vi "UNITTEST-JSON-RPC-Parse-Error.vi"(8 "error in (no error)":errorcluster) -> (0 "error out":errorcluster)   [LabVIEW 2019]
uses:
  <vilib>/addons/_JKI Toolkits/Caraya/classes/Assert/Assert Not Error.vi
  <vilib>/addons/_JKI Toolkits/Caraya/classes/Assert/Assert False.vi
  JSON-RPC/JSON-RPC.lvlib
  <vilib>/addons/_JKI Toolkits/Caraya/classes/Assert/Assert.lvclass
  <vilib>/addons/_JKI Toolkits/Caraya/classes/Test/Test.lvclass
  <vilib>/JDP Science/JSONtext/JSONtext.lvlib
panel:
  out "Array":string[](array[string])
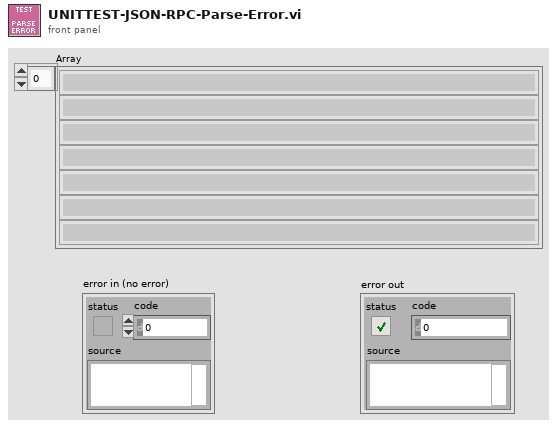
[diagram p1: front panel]
types:
  T1 = cluster{"error in (no error)":errorcluster, "id":string, "<JSON>":string, "response":string}[]
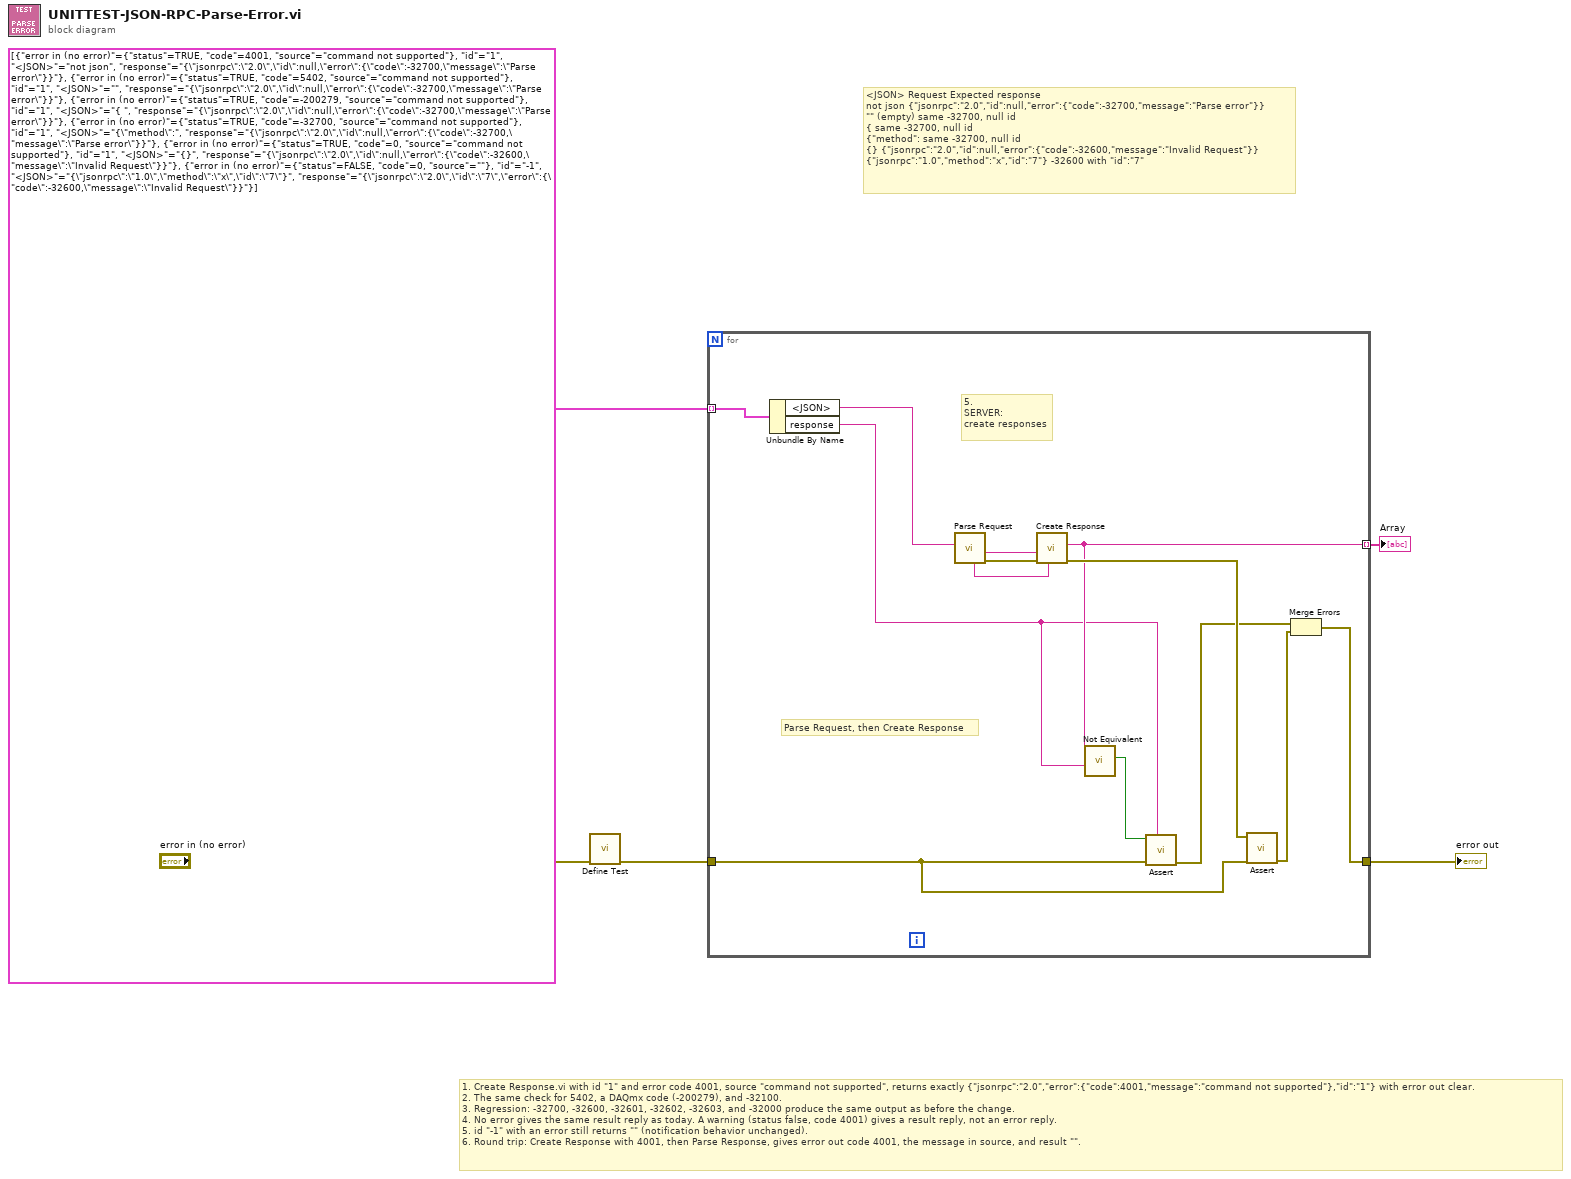
[diagram p0: block diagram]
diagram:
  # "<JSON> Request\tExpected response\nnot json\t{\"jsonrpc\":\"2.0\",\"id\":null,\"error\":{\"code\":-32700,\"message\":\"Parse error\"}}\n\"\" (empty)\tsame -32700, null id\n{\tsame -32700, null id\n{\"method\":\tsame -32700, null id\n{}\t{\"jsonrpc\":\"2.0\",\"id\":null,\"error\":{\"code\":-32600,\"message\":\"Invalid Request\"}}\n{\"jsonrpc\":\"1.0\",\"method\":\"x\",\"id\":\"7\"}\t-32600 with \"id\":\"7\""
  # "1. Create Response.vi with id \"1\" and error code 4001, source \"command not supported\", returns exactly {\"jsonrpc\":\"2.0\",\"error\":{\"code\":4001,\"message\":\"command not supported\"},\"id\":\"1\"} with error out clear.\n2. The same check for 5402, a DAQmx code (-200279), and -32100.\n3. Regression: -32700, -32600, -32601, -32602, -32603, and -32000 produce the same output as before the change.\n4. No error gives the same result reply as today. A warning (status false, code 4001) gives a result reply, not an error reply.\n5. id \"-1\" with an error still returns \"\" (notification behavior unchanged).\n6. Round trip: Create Response with 4001, then Parse Response, gives error out code 4001, the message in source, and result \"\"."
  n1 = call <vilib>:"Define Test.vi"("error in (no error)"="error in (no error)") -> ("error out"=w4:errorcluster)  [unwired: 9 in, 1 out]
  n2 = for {
    tunnel: [w12] -> w3 mode=indexing
    tunnel: w4 -> [w17]
    tunnel: [w14] -> w1
    tunnel: T1 [{"error in (no error)"={"status"=TRUE, "code"=4001, "source"="command not supported"}, "id"="1", "<JSON>"="not json", "response"="{\"jsonrpc\":\"2.0\",\"id\":null,\"error\":{\"code\":-32700,\"message\":\"Parse error\"}}"}, {"error in (no error)"={"status"=TRUE, "code"=5402, "source"="command not supported"}, "id"="1", "<JSON>"="", "response"="{\"jsonrpc\":\"2.0\",\"id\":null,\"error\":{\"code\":-32700,\"message\":\"Parse error\"}}"}, {"error in (no error)"={"status"=TRUE, "code"=-200279, "source"="command not supported"}, "id"="1", "<JSON>"="{ ", "response"="{\"jsonrpc\":\"2.0\",\"id\":null,\"error\":{\"code\":-32700,\"message\":\"Parse error\"}}"}, {"error in (no error)"={"status"=TRUE, "code"=-32700, "source"="command not supported"}, "id"="1", "<JSON>"="{\"method\":", "response"="{\"jsonrpc\":\"2.0\",\"id\":null,\"error\":{\"code\":-32700,\"message\":\"Parse error\"}}"}, {"error in (no error)"={"status"=TRUE, "code"=0, "source"="command not supported"}, "id"="1", "<JSON>"="{}", "response"="{\"jsonrpc\":\"2.0\",\"id\":null,\"error\":{\"code\":-32600,\"message\":\"Invalid Request\"}}"}, {"error in (no error)"={"status"=FALSE, "code"=0, "source"=""}, "id"="-1", "<JSON>"="{\"jsonrpc\":\"1.0\",\"method\":\"x\",\"id\":\"7\"}", "response"="{\"jsonrpc\":\"2.0\",\"id\":\"7\",\"error\":{\"code\":-32600,\"message\":\"Invalid Request\"}}"}] -> [w13] mode=indexing
    # "Parse Request, then Create Response"
    # "5.\nSERVER:\ncreate responses"
    n3 = Unbundle By Name(w13) -> ("<JSON>"=w9:string, "response"=w6:string)
    n4 = call "Parse Request.vi"("<JSON> Requests"=w9) -> ("error out"=w10:errorcluster, "Params"=w8:string, "IDs"=w7:string)  [unwired: 7 in, 1 out]
    n5 = call "Create Response.vi"("id"=w7, "error in (no error)"=w10, "result"=w8) -> ("error out"=w18:errorcluster, "<JSON> Response"=w12:string)  [unwired: 7 in]
    n6 = call <vilib>:"Not Equivalent.vi"("Other JSON"=w6, "JSON"=w12) -> ("Not Equivalent"=w11:bool)  [unwired: 8 in]
    n7 = call-poly <vilib>:"Assert.vi"("Label"=w6, "error in (no error)"=w17, "False?"=w11) -> ("error out"=w16:errorcluster)  [unwired: 7 in, 1 out]
    n8 = call-poly <vilib>:"Assert.vi"("error in (no error)"=w17, "Not Error?"=w18) -> ("error out"=w15:errorcluster)  [unwired: 8 in, 1 out]
    n9 = Merge Errors(w16, w15) -> (w14:errorcluster)
  }
  "error out" <- w1
  "Array" <- w3
